vi "Create Buffer.vi"(7 "Buffer Size (10k)":i32=10000 format="%.0p", 8 "error in (no error)":errorcluster, 11 "UI GUID":string) -> (0 "error out":errorcluster)   [LabVIEW 2025, in "CAN-LIN Raw Bus Capture UI.lvlib"]
uses:
  CAN-LIN Raw Bus Capture UI.lvlib
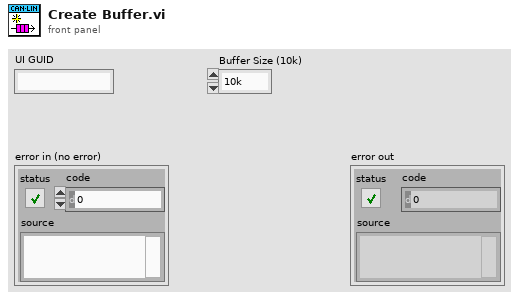
[diagram p1: front panel]
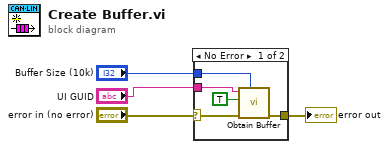
[diagram p0: block diagram]
diagram:
  n1 = case shown="No Error" "error in (no error)" {
    selector: "error in (no error)" -> [w8 w10]
    tunnel: [w9 w10] -> w3
    tunnel: "Buffer Size (10k)" -> [w6 _]
    tunnel: "UI GUID" -> [w5 _]
    frame No Error {
      n2 = call "Obtain Buffer.vi"("Buffer Size (10k)"=w6, "error in (no error)"=w8, "Create (F)"=TRUE ("create if not found? (T)"), "UI GUID"=w5) -> ("error out"=w9:errorcluster)  [unwired: 6 in, 1 out]
    }
    frame Error {
    }
  }
  "error out" <- w3
